vi "AddViToProject.vi"(5 "PropertyFolderName":string, 6 "ClassRef":refnum<vi>, 7 "Property":string, 8 "error out 2":errorcluster, 9 "PropertyNode":bool, 10 "NewVIPath":path, 11 "ProjectFolder":refnum<vi>) -> (0 "error out":errorcluster, 3 "AddFile":refnum<vi>)   [LabVIEW 2020, in "ClassWriterNative.lvclass"]
uses:
  ClassWriterNative.lvclass
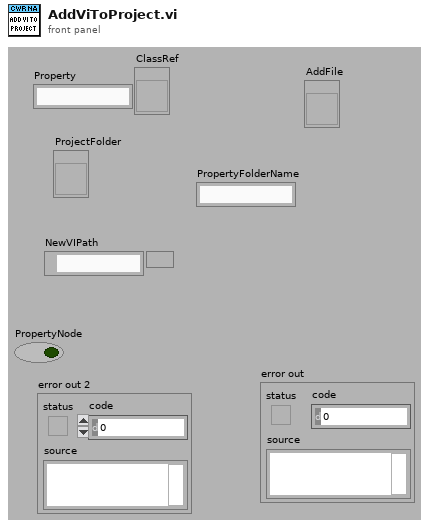
[diagram p1: front panel]
types:
  T1 = enum32{"invalid scope", "public", "private", "protected", "community"}
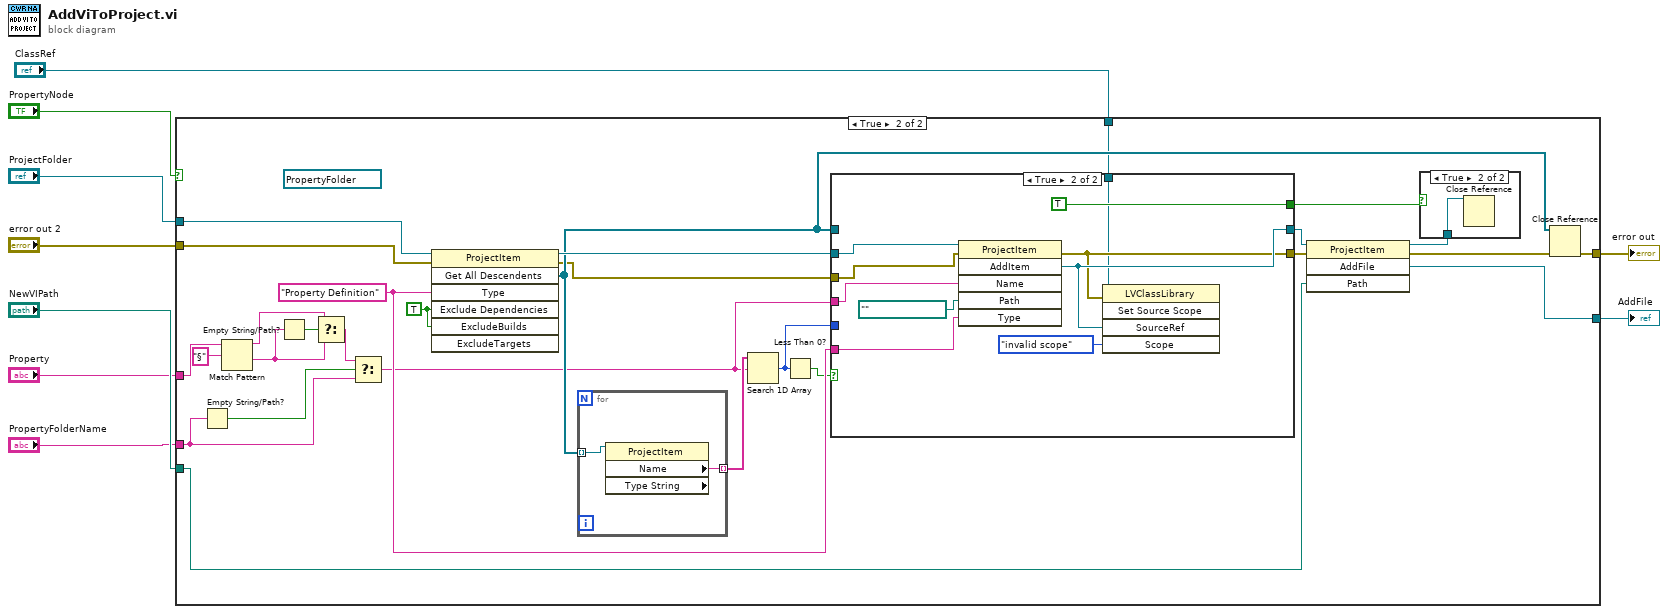
[diagram p0: block diagram]
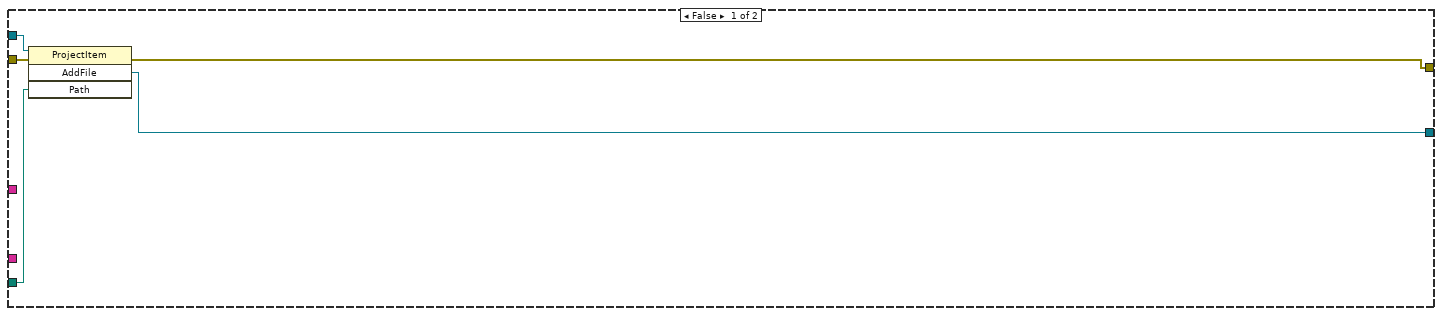
[diagram p2: hidden frame]
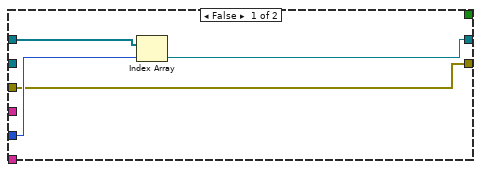
[diagram p4: hidden frame]
diagram:
  n1 = case shown="True" "PropertyNode" {
    tunnel: "ProjectFolder" -> [w14 w40]
    tunnel: "NewVIPath" -> [w13 w34]
    tunnel: "error out 2" -> [w12 w41]
    tunnel: [w11 w33] -> w8
    tunnel: [w10 w27] -> w2
    tunnel: "Property" -> [_ w29]
    tunnel: "PropertyFolderName" -> [_ w25]
    tunnel: "ClassRef" -> [_ w15]
    frame False {
      n2 = invoke class="ProjectItem" method="AddFile"(reference=w14, error in=w12, "Path"=w13) -> (error out=w10:errorcluster, "AddFile"=w11:refnum<vi>)  [unwired: 1 in, 2 out]
    }
    frame True {
      (unwired) refnum<vi> refnum ("reference out")
      w42 = TRUE ("ExcludeDependencies")
      w37 = "Property Definition" ("Type")
      n3 = Empty String/Path?(string/path=w25) -> (empty?=w26:bool)
      n4 = Match Pattern(string=w29, regular expression="§") -> (before substring=w19:string, after substring=w16:string)  [unwired: 1 in, 2 out]
      n5 = Empty String/Path?(string/path=w16) -> (empty?=w18:bool)
      n6 = Select(t=w19, s=w18, f=w16) -> (s? t:f=w17:string)
      n7 = Select(t=w17, s=w26, f=w25) -> (s? t:f=w24:string)
      n8 = invoke class="ProjectItem" method="Get All Descendents"(reference=w40, error in=w41, "Type"=w37, "Exclude Dependencies"=w42, "ExcludeBuilds"=w42) -> (reference out=w38:refnum<vi>, error out=w22:errorcluster, "All Descendents"=w31:refnum<vi>[])  [unwired: 2 in, 4 out]
      n9 = for {
        tunnel: w31 -> [w59] mode=indexing
        tunnel: [w58] -> w39 mode=indexing
        n10 = property class="ProjectItem" props=["Name", "Type String"](reference=w59) -> ("Name"=w58:string)  [unwired: 1 in, 3 out]
      }
      n11 = Search 1D Array(1D array=w39, element=w24) -> (index of element=w23:i32)  [unwired: 1 in]
      n12 = Less Than 0?(x=w23) -> (x < 0?=w28:bool)
      n13 = case shown="True" w28 {
        tunnel: w38 -> [_ w57]
        tunnel: w24 -> [_ w56]
        tunnel: w37 -> [_ w54]
        tunnel: [w46 w51] -> w36
        tunnel: [w44 w49] -> w35
        tunnel: w31 -> [w47 _]
        tunnel: w23 -> [w45 _]
        tunnel: w22 -> [w44 w53]
        tunnel: [_ TRUE] -> w21
        tunnel: w15 -> [_ w48]
        frame False {
          n14 = Index Array(array=w47, index=w45) -> (element=w46:refnum<vi>)
        }
        frame True {
          n15 = invoke class="ProjectItem" method="AddItem"(reference=w57, error in=w53, "Name"=w56, "Path"=path "", "Type"=w54) -> (error out=w49:errorcluster, "AddItem"=w51:refnum<vi>)  [unwired: 1 in, 4 out]
          n16 = invoke class="LVClassLibrary" method="Set Source Scope"(reference=w48, error in=w49, "SourceRef"=w51, "Scope"=T1."invalid scope" ("scope")) -> ()  [unwired: 1 in, 5 out]
        }
      }
      n17 = invoke class="ProjectItem" method="AddFile"(reference=w36, error in=w35, "Path"=w34) -> (reference out=w20:refnum<vi>, error out=w32:errorcluster, "AddFile"=w33:refnum<vi>)  [unwired: 1 in, 1 out]
      n18 = case shown="True" w21 {
        tunnel: w20 -> [_ w43]
        frame False {
        }
        frame True {
          n19 = Close Reference(reference=w43) -> ()  [unwired: 1 in, 1 out]
        }
      }
      n20 = Close Reference(reference=w31, error in (no error)=w32) -> (error out=w27:errorcluster)
    }
  }
  "error out" <- w2
  "AddFile" <- w8
